vi "remove Line Feed Const.vi"(10 "Input":string) -> (2 "Output":string)   [LabVIEW 2023, in "Spectrum Analyzer.lvlib" / "FSV-40N.lvclass"]
uses:
  FSV-40N.lvclass
  FSV-40N.lvclass/FSV-40N.ctl
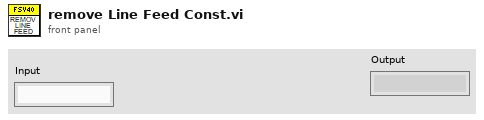
[diagram p1: front panel]
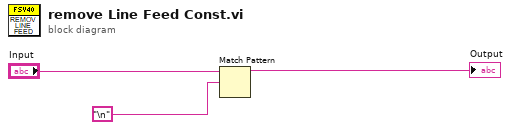
[diagram p0: block diagram]
diagram:
  n1 = Match Pattern(string="Input", regular expression="\n") -> (before substring=→"Output":string)  [unwired: 1 in, 3 out]
